vi "Get Available Enumerations.vi"(8 "error in (no error)":errorcluster, 10 "Feature":string, 11 "Camera in":refnum<class "Camera.lvclass">) -> (0 "error out":errorcluster, 2 "Available Enumerations":string[](array[string]), 3 "Camera":refnum<class "Camera.lvclass">)   [LabVIEW 2020, in "Camera.lvclass"]
uses:
  Camera.lvclass
  Camera.lvclass/Camera.ctl
  bin/gindustrialcam_32-1.dll
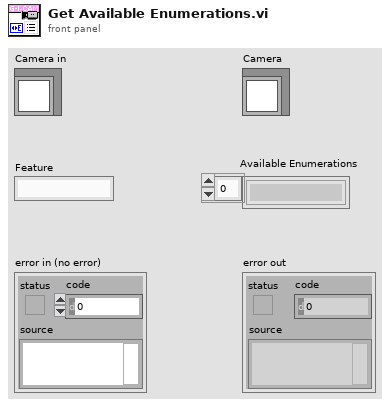
[diagram p1: front panel]
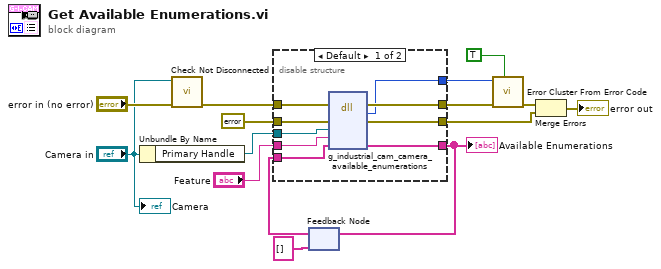
[diagram p0: block diagram]
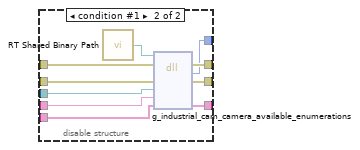
[diagram p2: hidden frame]
diagram:
  n1 = Unbundle By Name("Camera in") -> ("Primary Handle"=w4:refnum<data-value>)
  n2 = call "Check Not Disconnected.vi"("error in (no error)"="error in (no error)", "Camera in"="Camera in") -> ("error out"=w3:errorcluster)  [unwired: 9 in]
  n3 = feedback #1(string[] []) -> (w6:string[])
  n4 = disable-structure shown="Default" {
    disable-tunnel: [w24 w34] -> w13
    disable-tunnel: [w23 w33] -> w12
    disable-tunnel: [w22 w32] -> w10
    disable-tunnel: errorcluster {"status"=FALSE, "code"=0, "source"=""} ("error constant") -> [w21 w31]
    disable-tunnel: w6 -> [w20 w30]
    disable-tunnel: [w19 w29] -> w5
    disable-tunnel: w4 -> [w18 w28]
    disable-tunnel: w3 -> [w17 w27]
    disable-tunnel: "Feature" -> [w16 w26]
    frame condition #0 (active) {
      n5 = dll-call lib="C:/serenial/lib/g-industrial-camera/LabVIEW/g_industrial_cam/bin/gindustrialcam_*-1.*" fn="g_industrial_cam_camera_available_enumerations"(error in=w17, "err"=w21, "edvr"=w18, "feature"=w16, "enum values"=w20) -> (error out=w24:errorcluster, "Mg_Error"=w23:i32, "err"=w22:errorcluster, "enum values"=w19:string[])  [unwired: 4 in, 1 out]
    }
    frame condition #1 {
      n6 = call "RT Shared Binary Path.vi"() -> ("Path"=w25:path)
      n7 = dll-call lib="C:/serenial/lib/g-industrial-camera/LabVIEW/g_industrial_cam/bin/gindustrialcam_*-1.*" fn="g_industrial_cam_camera_available_enumerations"(path in=w25, error in=w27, "err"=w31, "edvr"=w28, "feature"=w26, "enum values"=w30) -> (error out=w34:errorcluster, "Mg_Error"=w33:i32, "err"=w32:errorcluster, "enum values"=w29:string[])  [unwired: 3 in, 1 out]
    }
  }
  "Available Enumerations" <- w5
  n8 = feedback-in #1(w5) -> ()
  n9 = call <vilib>:"Error Cluster From Error Code.vi"("show call chain? (False)"=TRUE, "error in (no error)"=w13, "error code (0)"=w12) -> ("error out"=w11:errorcluster)  [unwired: 6 in]
  n10 = Merge Errors(w11, w10) -> (→"error out":errorcluster)
  "Camera" <- "Camera in"
